vi "Convert String Register Value.vi"(8 "error in (no error)":errorcluster, 10 "Register Values":u16[](array[numeric]) format="%04x", 11 "Modbus in":refnum<class "Modbus.lvclass">) -> (0 "error out":errorcluster, 2 "String out":string, 3 "Modbus out":refnum<class "Modbus.lvclass">)   [LabVIEW 2026, in "Modbus.lvlib" / "Modbus.lvclass"]
uses:
  Modbus.lvclass
  Modbus.lvclass/Modbus.ctl
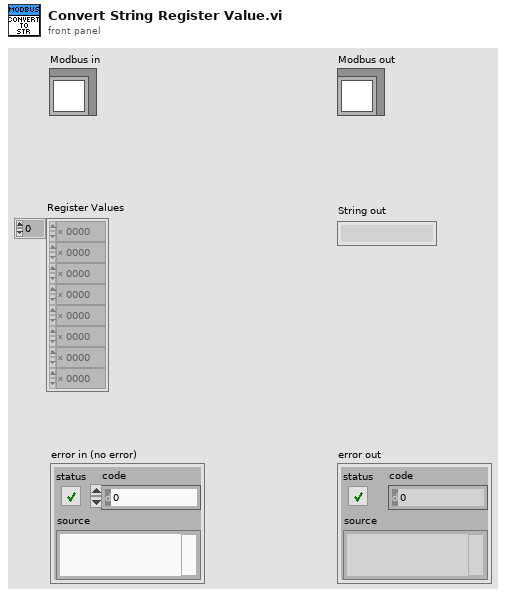
[diagram p1: front panel]
types:
  T1 = typedef "Modbus.lvlib/Modbus.lvclass/Order.ctl" = enum16{"Big-Endian (AB CD)", "Word-Swap (CD AB)", "Byte-Swap (BA DC)", "Little-Endian (DC BA)"}
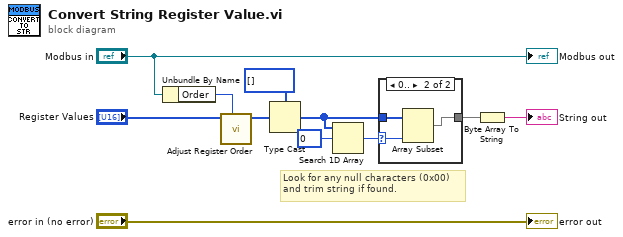
[diagram p0: block diagram]
diagram:
  # "Look for any null characters (0x00)\nand trim string if found."
  n1 = Unbundle By Name("Modbus in") -> ("Order"=w1:T1)
  n2 = call "Adjust Register Order.vi"("Order"=w1, "Register Values in"="Register Values") -> ("Register Values out"=w9:u16[])  [unwired: 9 in]
  n3 = Type Cast(type=u8[] [], x=w9) -> (*(type *) &x=w7:u8[])
  n4 = Search 1D Array(1D array=w7, element=u8 0) -> (index of element=w4:i32)  [unwired: 1 in]
  n5 = case shown="0.." w4 {
    selector: w4 -> [_ w13]
    tunnel: w7 -> [w12 w15]
    tunnel: [w12 w14] -> w6
    frame Default {
    }
    frame 0.. {
      n6 = Array Subset(array=w15, length=w13) -> (w14:u8[])  [unwired: 1 in]
    }
  }
  n7 = Byte Array To String(unsigned byte array=w6) -> (string=→"String out":string)
  "Modbus out" <- "Modbus in"
  "error out" <- "error in (no error)"
